vi "Close.vi"(8 "error in (no error)":errorcluster, 10 "Reason":T1, 11 "Panel in":refnum<class "Panel.lvclass">) -> (0 "error out":errorcluster, 3 "Panel out":refnum<class "Panel.lvclass">)   [LabVIEW 2020, in "OOPanel.lvlib" / "Panel.lvclass"]
uses:
  Panel.lvclass
  Close Reason.ctl
  Panel.lvclass/Panel.ctl
  OOPanel.lvlib
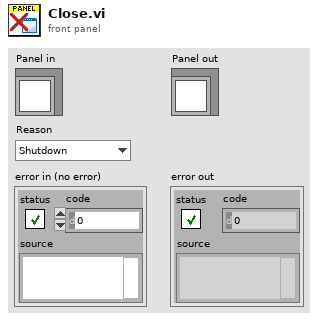
[diagram p1: front panel]
types:
  T1 = typedef "OOPanel.lvlib/Close Reason.ctl" = enum16{"Shutdown", "Close"}
  T2 = typedef "OOPanel.lvlib/Panel.lvclass/Ref Data.ctl" = cluster{"Panel Ref":refnum<vi>, "SubPanel":refnum<vi>, "Close":bool, "Running":bool, "State":T3}
  T3 = typedef "OOPanel.lvlib/Visibility State.ctl" = enum16{"Idle", "Closed", "Hidden", "Visible", "Subpanel", "Hidden Subpanel"}
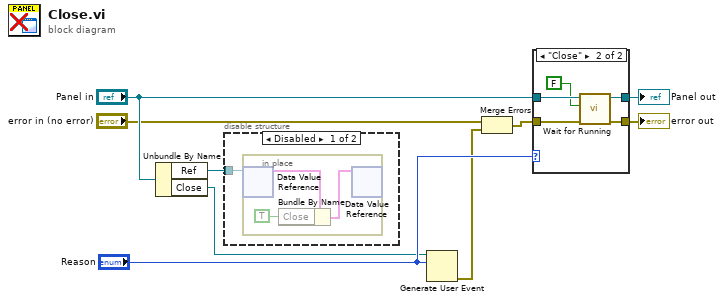
[diagram p0: block diagram]
diagram:
  n1 = Unbundle By Name("Panel in") -> ("Ref"=w9:refnum<data-value>, "Close"=w3:refnum<user-event>)
  n2 = disable-structure shown="Disabled" {
    disable-tunnel: w9 -> [w10 _]
    frame Disabled {
      n3 = in-place {
        n4 = in-place-dvr #1(w10) -> (w13:T2)  [unwired: 1 out]
        n5 = Bundle By Name(cluster=w13, "Close"=TRUE) -> (w11:T2)
        n6 = in-place-dvr #1(w11) -> ()  [unwired: 2 out]
      }
    }
    frame Enabled {
    }
  }
  n7 = Generate User Event(user event=w3, event data cluster="Reason") -> (error out=w1:errorcluster)  [unwired: 2 in, 1 out]
  n8 = Merge Errors("error in (no error)", w1) -> (w2:errorcluster)
  n9 = case shown="\"Close\"" "Reason" {
    tunnel: "Panel in" -> [w15 w20]
    tunnel: w2 -> [w14 w19]
    tunnel: [w14 w17] -> w6
    tunnel: [w15 w16] -> w5
    frame "Shutdown" {
    }
    frame "Close" {
      n10 = call "Wait for Running.vi"("error in (no error)"=w19, "Running"=FALSE, "Panel in"=w20) -> ("error out"=w17:errorcluster, "Panel out"=w16:refnum<class "Panel.lvclass">)  [unwired: 7 in]
    }
  }
  "error out" <- w6
  "Panel out" <- w5
